vi "Build DS OpModes.vi"(6 "utility names":string[](array[string]), 8 "error in (no error)":errorcluster, 9 "tele names":string[](array[string])=["TeleOp"], 11 "auto names":string[](array[string])=["Auto"]) -> (0 "error in (no error) 2":errorcluster)   [LabVIEW 2023, in "MrcLib.lvlib"]
doc: "Simple way to update OpModes with named choices."
uses:
  <vilib>/MRC/MrcLib.lvlib
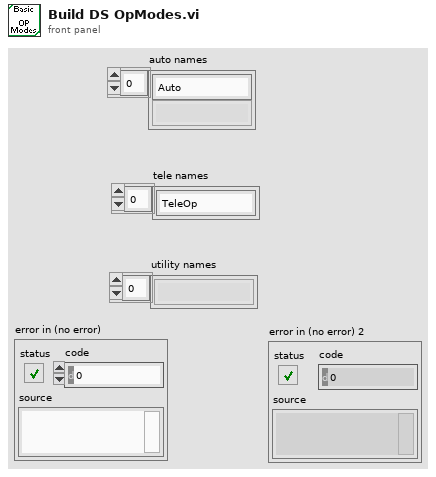
[diagram p1: front panel]
types:
  T1 = cluster{"hash":u64, "name":string, "group":string, "description":string, "text color":u32, "BG color":u32}
  T2 = cluster{"hash":u64, "name":string, "group":string, "description":string, "text color":u32, "BG color":u32}[]
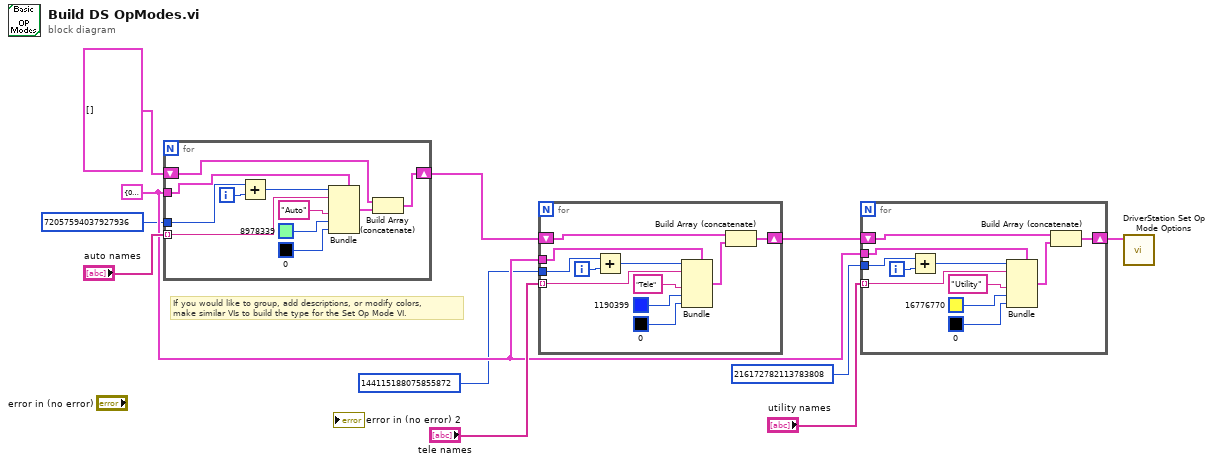
[diagram p0: block diagram]
diagram:
  w4 = T1 {"hash"=0, "name"="", "group"="", "description"="", "text color"=0, "BG color"=0} ("opModes out 2")
  # "If you would like to group, add descriptions, or modify colors,\nmake similar VIs to build the type for the Set Op Mode VI."
  n1 = for {
    tunnel: "auto names" -> [w21] mode=indexing
    shift-right: [w18] -> w8
    shift-left: T2 [] ("OpModes") -> [w17]
    tunnel: w4 -> [w22]
    tunnel: u64 72057594037927936 ("hash") -> [w15]
    i -> [w14]
    n2 = Add(x=w15, y=w14) -> (x+y=w13:u64)
    n3 = Bundle(cluster=w22, "hash"=w13, "name"=w21, "description"="Auto" ("group"), "text color"=u32 8978339, "BG color"=u32 0) -> (w16:T1)  [unwired: 1 in]
    n4 = Build Array (concatenate)(w17, w16) -> (w18:T2)
  }
  n5 = for {
    tunnel: "tele names" -> [w30] mode=indexing
    shift-right: [w29] -> w7
    shift-left: w8 -> [w27]
    tunnel: w4 -> [w31]
    tunnel: u64 144115188075855872 ("hash") -> [w24]
    i -> [w26]
    n6 = Add(x=w24, y=w26) -> (x+y=w25:u64)
    n7 = Bundle(cluster=w31, "hash"=w25, "name"=w30, "description"="Tele" ("group"), "text color"=u32 1190399, "BG color"=u32 0) -> (w28:T1)  [unwired: 1 in]
    n8 = Build Array (concatenate)(w27, w28) -> (w29:T2)
  }
  n9 = for {
    tunnel: "utility names" -> [w41] mode=indexing
    shift-right: [w38] -> w6
    shift-left: w7 -> [w40]
    tunnel: w4 -> [w42]
    tunnel: u64 216172782113783808 ("hash") -> [w37]
    i -> [w35]
    n10 = Add(x=w37, y=w35) -> (x+y=w36:u64)
    n11 = Bundle(cluster=w42, "hash"=w36, "name"=w41, "description"="Utility", "text color"=u32 16776770, "BG color"=u32 0) -> (w39:T1)  [unwired: 1 in]
    n12 = Build Array (concatenate)(w40, w39) -> (w38:T2)
  }
  n13 = call <vilib>:"DriverStation Set Op Mode Options.vi"("opModes"=w6) -> ()  [unwired: 10 in, 1 out]
